vi "Go to 0 with Return Speed.vi"(8 "error in (no error)":errorcluster, 11 "AUDIX EM1000 in":refnum<class "AUDIX EM1000.lvclass">) -> (0 "error out":errorcluster, 1 "Final Speed":i32, 2 "Return Speed":i32, 3 "AUDIX EM1000 out":refnum<class "AUDIX EM1000.lvclass">, 4 "TT Angle":dbl)   [LabVIEW 2023, in "Turn Table and Mast.lvlib" / "AUDIX EM1000.lvclass"]
uses:
  AUDIX EM1000.lvclass
  AUDIX EM1000.lvclass/AUDIX EM1000.ctl
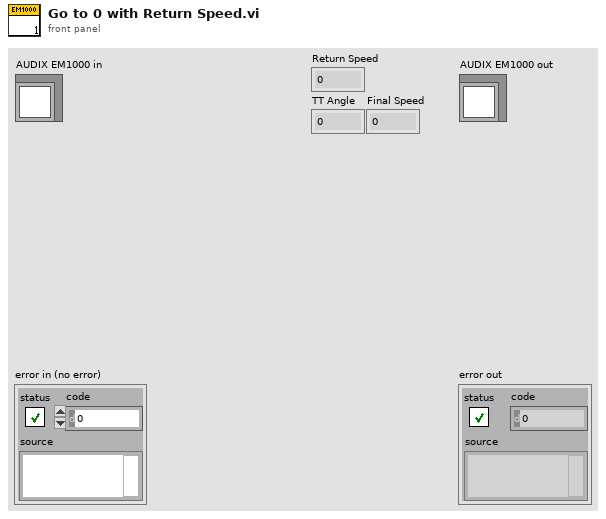
[diagram p1: front panel]
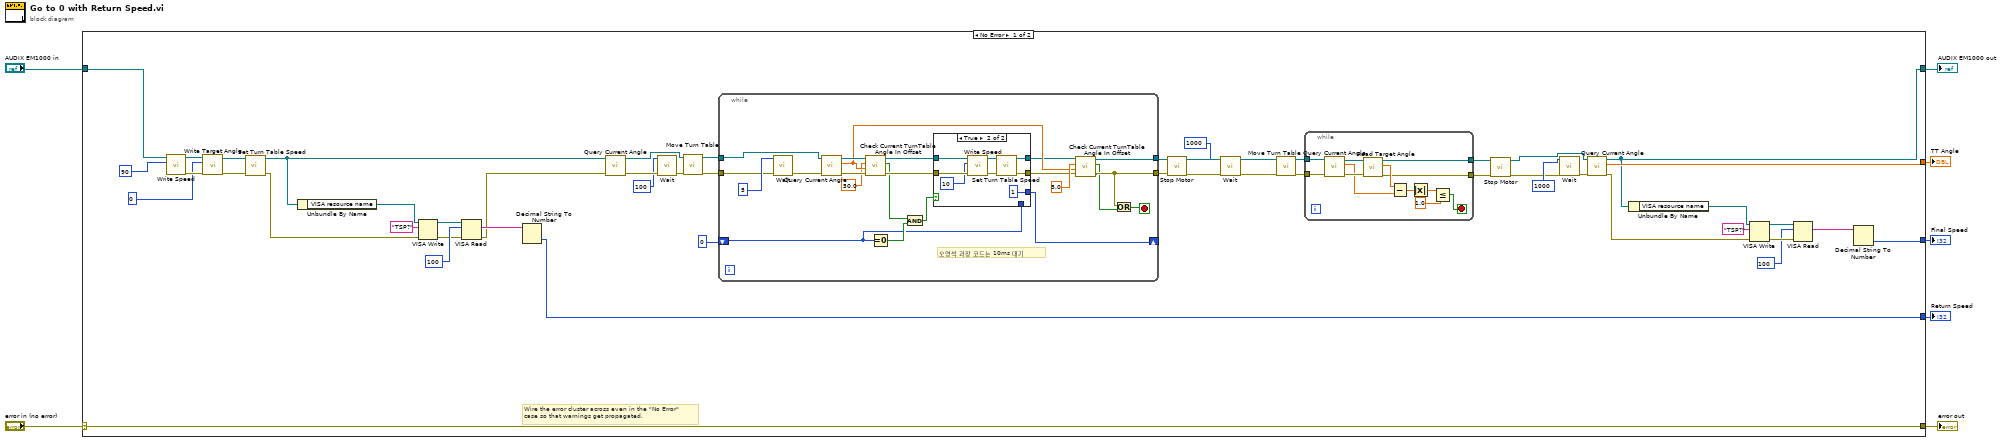
[diagram p0: block diagram]
diagram:
  n1 = case shown="No Error" "error in (no error)" {
    selector: "error in (no error)" -> [w56 w103]
    tunnel: [w56 w103] -> w6
    tunnel: [w18 w102] -> w4
    tunnel: "AUDIX EM1000 in" -> [w40 w102]
    tunnel: [w28 _] -> w3
    tunnel: [w27 _] -> w2
    tunnel: [w19 _] -> w1
    frame No Error {
      # "Wire the error cluster across even in the \"No Error\"\ncase so that warnings get propagated."
      n2 = call "Write Speed.vi"("Speed"=90, "AUDIX EM1000 in"=w40) -> ("error out"=w52:errorcluster, "AUDIX EM1000 out"=w53:refnum<class "AUDIX EM1000.lvclass">)  [unwired: 8 in]
      n3 = call "Write Target Angle.vi"("error in (no error)"=w52, "Target Angle"=0, "AUDIX EM1000 in"=w53) -> ("error out"=w42:errorcluster, "AUDIX EM1000 out"=w43:refnum<class "AUDIX EM1000.lvclass">)  [unwired: 7 in]
      n4 = call-dynamic "Set Turn Table Speed.vi"("error in (no error)"=w42, "AUDIX EM1000 in"=w43) -> ("error out"=w30:errorcluster, "AUDIX EM1000 out"=w37:refnum<class "AUDIX EM1000.lvclass">)  [unwired: 8 in]
      n5 = Unbundle By Name(w37) -> ("VISA resource name"=w31:refnum<visa-resource-name>)
      n6 = VISA Write(VISA resource name=w31, write buffer="TSP?", error in (no error)=w30) -> (VISA resource name out=w35:refnum<visa-resource-name>, error out=w33:errorcluster)  [unwired: 1 out]
      n7 = VISA Read(VISA resource name=w35, byte count=u32 100, error in (no error)=w33) -> (read buffer=w32:string, error out=w29:errorcluster)  [unwired: 2 out]
      n8 = Decimal String To Number(string=w32) -> (number=w28:i32)  [unwired: 2 in, 1 out]
      n9 = call-dynamic "Query Current Angle.vi"("error in (no error)"=w29, "AUDIX EM1000 in"=w37) -> ("error out"=w45:errorcluster, "AUDIX EM1000 out"=w46:refnum<class "AUDIX EM1000.lvclass">)  [unwired: 7 in, 1 out]
      n10 = call "Wait.vi"("에러 상수 입력"=w45, "대기 시간 (ms)"=u32 100) -> ("에러 상수 출력"=w47:errorcluster)  [unwired: 9 in]
      n11 = call-dynamic "Move Turn Table.vi"("error in (no error)"=w47, "AUDIX EM1000 in"=w46) -> ("error out"=w54:errorcluster, "AUDIX EM1000 out"=w55:refnum<class "AUDIX EM1000.lvclass">)  [unwired: 8 in]
      n12 = while {
        tunnel: w55 -> [w89]
        tunnel: [w85] -> w50
        tunnel: [w82] -> w51
        tunnel: w54 -> [w86]
        shift-right: [w70] -> _
        shift-left: 0 -> [w69]
        stop <- w87 stop-if-true
        # "오영석 과장 코드는 10ms 대기"
        n13 = call "Wait.vi"("에러 상수 입력"=w86, "대기 시간 (ms)"=u32 5) -> ("에러 상수 출력"=w88:errorcluster)  [unwired: 9 in]
        n14 = call-dynamic "Query Current Angle.vi"("error in (no error)"=w88, "AUDIX EM1000 in"=w89) -> ("error out"=w79:errorcluster, "Current Angle"=w80:dbl, "AUDIX EM1000 out"=w81:refnum<class "AUDIX EM1000.lvclass">)  [unwired: 7 in]
        n15 = call-dynamic "Check Current TurnTable Angle In Offset.vi"("error in (no error)"=w79, "Target Offset"=w80, "Current Angle"=50.0 ("Target Offset"), "AUDIX EM1000 in"=w81) -> ("error out"=w76:errorcluster, "In Offset Range?"=w72:bool, "AUDIX EM1000 out"=w77:refnum<class "AUDIX EM1000.lvclass">)  [unwired: 5 in]
        n16 = Equal To 0?(x=w69) -> (x = 0?=w73:bool)
        n17 = And(x=w72, y=w73) -> (x .and. y?=w71:bool)
        n18 = case shown="True" w71 {
          tunnel: w77 -> [w93 w96]
          tunnel: w76 -> [w92 w95]
          tunnel: [w93 w101] -> w75
          tunnel: [w92 w100] -> w74
          tunnel: [w91 1] -> w70
          tunnel: w69 -> [w91 _]
          frame False {
          }
          frame True {
            n19 = call "Write Speed.vi"("error in (no error)"=w95, "Speed"=10 ("Target Angle"), "AUDIX EM1000 in"=w96) -> ("error out"=w98:errorcluster, "AUDIX EM1000 out"=w97:refnum<class "AUDIX EM1000.lvclass">)  [unwired: 7 in]
            n20 = call-dynamic "Set Turn Table Speed.vi"("error in (no error)"=w98, "AUDIX EM1000 in"=w97) -> ("error out"=w100:errorcluster, "AUDIX EM1000 out"=w101:refnum<class "AUDIX EM1000.lvclass">)  [unwired: 8 in]
          }
        }
        n21 = call-dynamic "Check Current TurnTable Angle In Offset.vi"("error in (no error)"=w74, "Target Offset"=w80, "Current Angle"=5.0 ("Target Offset"), "AUDIX EM1000 in"=w75) -> ("error out"=w85:errorcluster, "In Offset Range?"=w84:bool, "AUDIX EM1000 out"=w82:refnum<class "AUDIX EM1000.lvclass">)  [unwired: 5 in]
        n22 = Or(x=w85, y=w84) -> (x .or. y?=w87:bool)
      }
      n23 = call-dynamic "Stop Motor.vi"("error in (no error)"=w50, "AUDIX EM1000 in"=w51) -> ("error out"=w10:errorcluster, "AUDIX EM1000 out"=w17:refnum<class "AUDIX EM1000.lvclass">)  [unwired: 8 in]
      n24 = call "Wait.vi"("에러 상수 입력"=w10, "대기 시간 (ms)"=u32 1000) -> ("에러 상수 출력"=w8:errorcluster)  [unwired: 9 in]
      n25 = call-dynamic "Move Turn Table.vi"("error in (no error)"=w8, "AUDIX EM1000 in"=w17) -> ("error out"=w15:errorcluster, "AUDIX EM1000 out"=w16:refnum<class "AUDIX EM1000.lvclass">)  [unwired: 8 in]
      n26 = while {
        tunnel: w16 -> [w68]
        tunnel: w15 -> [w67]
        tunnel: [w58] -> w14
        tunnel: [w57] -> w13
        stop <- w59 stop-if-true
        n27 = call-dynamic "Query Current Angle.vi"("error in (no error)"=w67, "AUDIX EM1000 in"=w68) -> ("error out"=w65:errorcluster, "Current Angle"=w63:dbl, "AUDIX EM1000 out"=w66:refnum<class "AUDIX EM1000.lvclass">)  [unwired: 7 in]
        n28 = call "Read Target Angle.vi"("error in (no error)"=w65, "AUDIX EM1000 in"=w66) -> ("error out"=w57:errorcluster, "Target Angle"=w64:dbl, "AUDIX EM1000 out"=w58:refnum<class "AUDIX EM1000.lvclass">)  [unwired: 7 in]
        n29 = Subtract(x=w64, y=w63) -> (x-y=w62:dbl)
        n30 = Absolute Value(x=w62) -> (abs(x)=w61:dbl)
        n31 = Less Or Equal?(x=w61, y=1.0) -> (x <= y?=w59:bool)
      }
      n32 = call-dynamic "Stop Motor.vi"("error in (no error)"=w13, "AUDIX EM1000 in"=w14) -> ("error out"=w12:errorcluster, "AUDIX EM1000 out"=w11:refnum<class "AUDIX EM1000.lvclass">)  [unwired: 8 in]
      n33 = call "Wait.vi"("에러 상수 입력"=w12, "대기 시간 (ms)"=u32 1000) -> ("에러 상수 출력"=w49:errorcluster)  [unwired: 9 in]
      n34 = call-dynamic "Query Current Angle.vi"("error in (no error)"=w49, "AUDIX EM1000 in"=w11) -> ("error out"=w20:errorcluster, "Current Angle"=w27:dbl, "AUDIX EM1000 out"=w18:refnum<class "AUDIX EM1000.lvclass">)  [unwired: 7 in]
      n35 = Unbundle By Name(w18) -> ("VISA resource name"=w26:refnum<visa-resource-name>)
      n36 = VISA Write(VISA resource name=w26, write buffer="TSP?", error in (no error)=w20) -> (VISA resource name out=w22:refnum<visa-resource-name>, error out=w24:errorcluster)  [unwired: 1 out]
      n37 = VISA Read(VISA resource name=w22, byte count=u32 100, error in (no error)=w24) -> (read buffer=w25:string)  [unwired: 3 out]
      n38 = Decimal String To Number(string=w25) -> (number=w19:i32)  [unwired: 2 in, 1 out]
    }
    frame Error {
    }
  }
  "error out" <- w6
  "AUDIX EM1000 out" <- w4
  "Return Speed" <- w3
  "TT Angle" <- w2
  "Final Speed" <- w1
